vi "Numeric Size to Register Quantity.vi"(1 "Size":T1) -> (0 "Quantity":u16)   [LabVIEW 2026, in "Modbus.lvlib" / "Modbus.lvclass"]
uses:
  Modbus.lvclass
  Types/Numeric Size.ctl
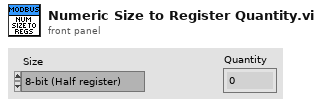
[diagram p1: front panel]
types:
  T1 = typedef "Modbus.lvlib/Modbus.lvclass/Numeric Size.ctl" = enum16{"8-bit (Half register)", "16-bit (One register)", "32-bit (Two registers)", "64-bit (Four registers)"}
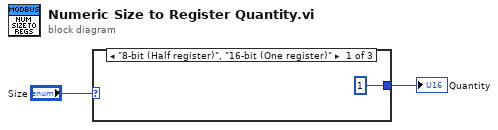
[diagram p0: block diagram]
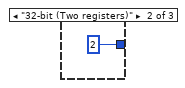
[diagram p2: hidden frame]
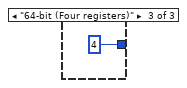
[diagram p3: hidden frame]
diagram:
  n1 = case shown="\"8-bit (Half register)\", \"16-bit (One register)\"" "Size" {
    tunnel: [u16 1 ("Quantity") u16 2 ("Quantity") u16 4 ("Quantity")] -> w1
    frame "8-bit (Half register)", "16-bit (One register)" {
    }
    frame "32-bit (Two registers)" {
    }
    frame "64-bit (Four registers)" {
    }
  }
  "Quantity" <- w1
